vi "Power Reset.vi"() -> (0 "error out":errorcluster, 2 "Result":string, 3 "Result":bool)   [LabVIEW 2021]
uses:
  10054_Control Folder/Support/Relay_no.ctl
panel:
  out "status":bool
  in  "error in (no error)":errorcluster
  out ".not. x?":bool
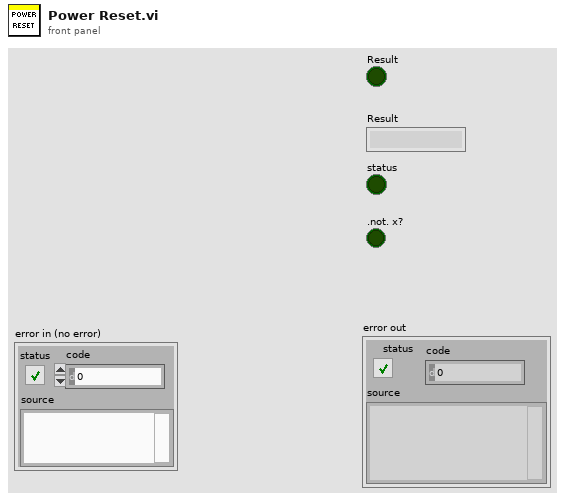
[diagram p1: front panel]
types:
  T1 = typedef "Relay_no.ctl" = enum16{"Init", "write&Read", "PCB Serial Write & Read", "PCB Write SSD & Password", "Read Wifi state", "Reset", "Close"}
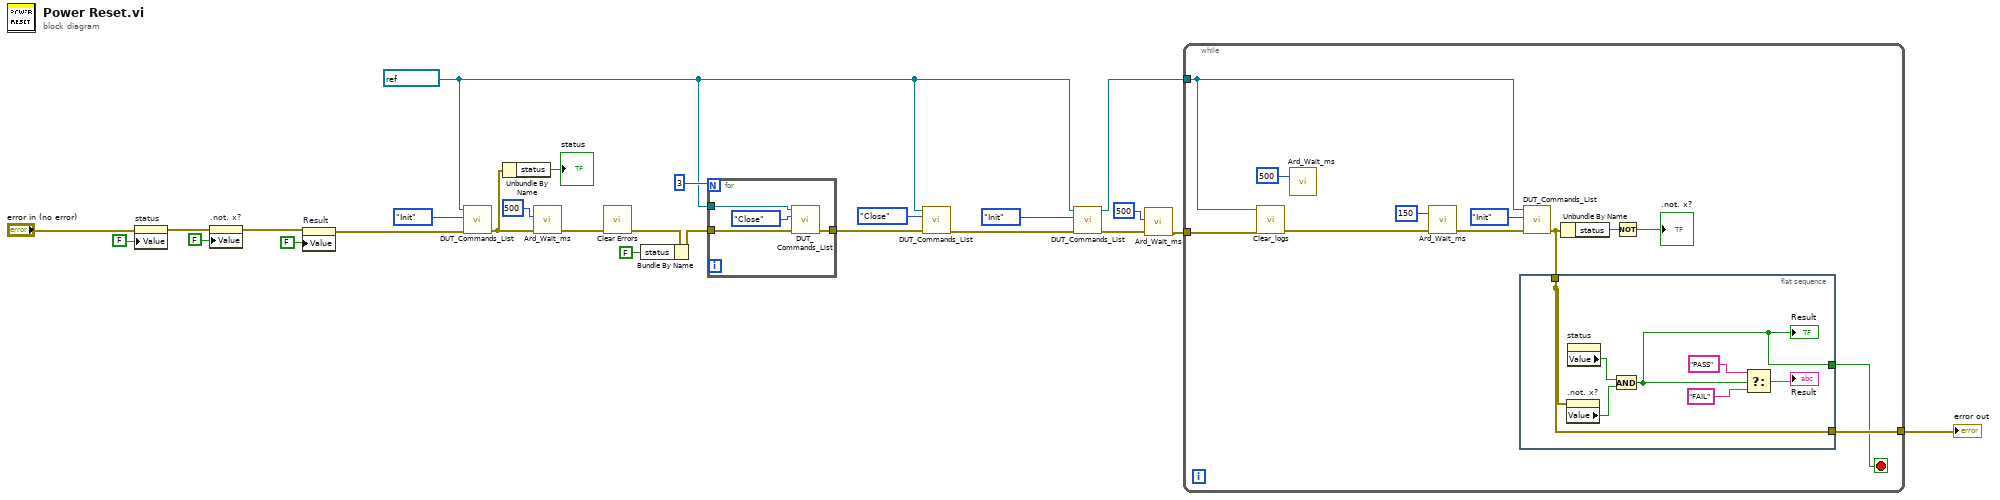
[diagram p0: block diagram]
diagram:
  w8 = refnum<visa-resource-name> "COM3" ("Resource In")
  n1 = property on="status" class="Bool (strict)"(error in="error in (no error)", "Value"=FALSE ("status")) -> (error out=w7:errorcluster)  [unwired: 1 in, 1 out]
  n2 = property on=".not. x?" class="Bool (strict)"(error in=w7, "Value"=FALSE (".not. x?")) -> (error out=w6:errorcluster)  [unwired: 1 in, 1 out]
  n3 = property on="Result" class="Bool (strict)"(error in=w6, "Value"=FALSE ("Result")) -> (error out=w5:errorcluster)  [unwired: 1 in, 1 out]
  n4 = call "DUT_Commands_List.vi"("error in"=w5, "Operation"=Relay_no."Init", "Resource In"=w8) -> ("error out"=w22:errorcluster)  [unwired: 6 in, 2 out]
  n5 = Unbundle By Name(w22) -> ("status"=→"status":bool)
  n6 = call "Ard_Wait_ms.vi"("error in"=w22, "millisec"=u32 500) -> ("error in 2"=w21:errorcluster)  [unwired: 9 in]
  n7 = call <vilib>:"Clear Errors.vi"("error in (no error)"=w21) -> ("error out"=w19:errorcluster)  [unwired: 5 in, 1 out]
  n8 = Bundle By Name(cluster=w19, "status"=FALSE) -> (w17:errorcluster)
  n9 = for {
    N: 3 -> [_]
    tunnel: w8 -> [w27]
    tunnel: w17 -> [w29]
    tunnel: [w28] -> w15
    n10 = call "DUT_Commands_List.vi"("error in"=w29, "Operation"=Relay_no."Close", "Resource In"=w27) -> ("error out"=w28:errorcluster)  [unwired: 6 in, 2 out]
  }
  n11 = call "DUT_Commands_List.vi"("error in"=w15, "Operation"=Relay_no."Close", "Resource In"=w8) -> ("error out"=w14:errorcluster)  [unwired: 6 in, 2 out]
  n12 = call "DUT_Commands_List.vi"("error in"=w14, "Operation"=Relay_no."Init", "Resource In"=w8) -> ("error out"=w10:errorcluster, "Resource out"=w1:refnum<visa-resource-name>)  [unwired: 6 in, 1 out]
  n13 = call "Ard_Wait_ms.vi"("error in"=w10, "millisec"=u32 500) -> ("error in 2"=w9:errorcluster)  [unwired: 9 in]
  n14 = while {
    tunnel: [w35] -> w26
    tunnel: w9 -> [w32]
    tunnel: w1 -> [w33]
    stop <- w34 stop-if-true
    n15 = call "Clear_logs.vi"("error in (no error)"=w32, "VISA resource name"=w33) -> ("error out"=w40:errorcluster)  [unwired: 6 in, 1 out]
    n16 = call "Ard_Wait_ms.vi"("millisec"=u32 500) -> ()  [unwired: 10 in, 1 out]
    n17 = call "Ard_Wait_ms.vi"("error in"=w40, "millisec"=u32 150) -> ("error in 2"=w41:errorcluster)  [unwired: 9 in]
    n18 = flat-sequence {
      tunnel: w36 -> [w45]
      tunnel: [w45] -> w35
      tunnel: [w44] -> w34
      frame #0 {
        n19 = property on=".not. x?" class="Bool (strict)"(error in=w45) -> ("Value"=w49:bool)  [unwired: 1 in, 2 out]
        n20 = property on="status" class="Bool (strict)"() -> ("Value"=w43:bool)  [unwired: 2 in, 2 out]
        n21 = And(x=w43, y=w49) -> (x .and. y?=w44:bool)
        "Result" <- w44
        n22 = Select(t="PASS", s=w44, f="FAIL") -> (s? t:f=→"Result":string)
      }
    }
    n23 = call "DUT_Commands_List.vi"("error in"=w41, "Operation"=Relay_no."Init", "Resource In"=w33) -> ("error out"=w36:errorcluster)  [unwired: 6 in, 2 out]
    n24 = Unbundle By Name(w36) -> ("status"=w38:bool)
    n25 = Not(x=w38) -> (.not. x?=→".not. x?":bool)
  }
  "error out" <- w26
